vi "RemoteVI Start Window.vi"(0 "window":u64, 1 "whole network?":bool, 2 "token":string, 3 "view only?":bool, 5 "port":u16=8100, 7 "fps":dbl=20.0, 8 "VI Server":string, 11 "error in":errorcluster) -> (4 "URL":string, 15 "error out":errorcluster)   [LabVIEW 2020, in "RemoteVI.lvlib"]
doc: "Shares a WINDOW of any process in a web browser - a front panel of another LabVIEW (a built application or another LabVIEW version), or a window of any other program - and returns immediately. window is its handle (HWND); RemoteVI Server lists the windows that can be shared. Everything else is as RemoteVI Start.vi: URL is the link with the access token, this computer only unless whole network? is TRUE, token empty makes a random one, view only? ignores the browsers' input, one share per port. A window target is streamed and operated through Win32 only: the picture, clicks, keys, menus and popups, and the dialogs and other windows of its process; tip strips and splitter dragging need the VI's own LabVIEW (VI Server) and are not available, and Shift, Ctrl and Alt reach another process only in the mouse messages' flags (docs\\architecture.md). The share stops on RemoteVI Stop.vi with the same port, or by itself when the window is closed."
uses:
  RemoteVI.lvlib
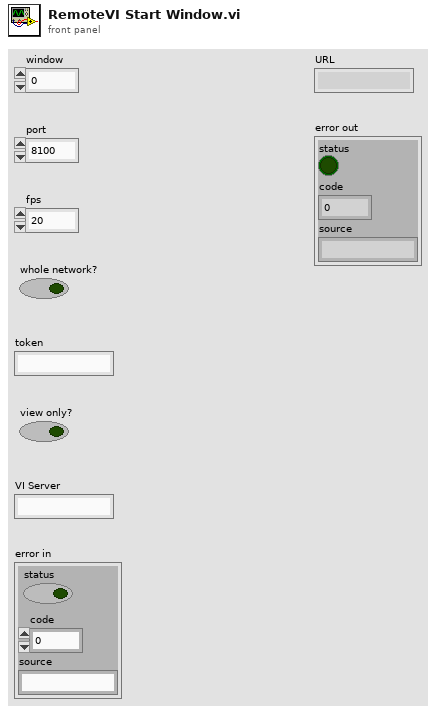
[diagram p1: front panel]
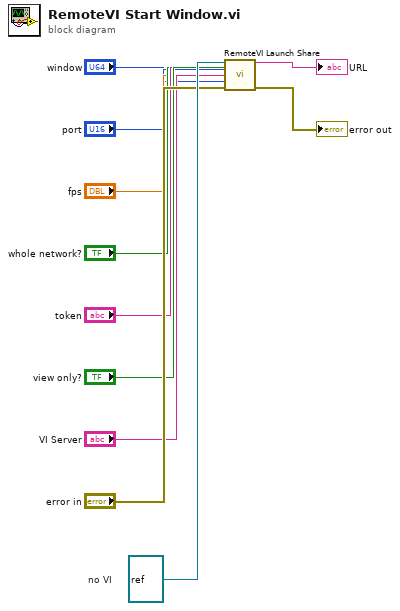
[diagram p0: block diagram]
diagram:
  w9 = refnum<vi> refnum  # no VI
  n1 = call "RemoteVI Launch Share.vi"("VI"=w9, "whole network?"="whole network?", "token"="token", "view only?"="view only?", "port"="port", "fps"="fps", "VI Server"="VI Server", "window"="window", "error in"="error in") -> ("URL"=→"URL":string, "error out"=→"error out":errorcluster)  [unwired: 5 in]
